vi "RemoteVI Send Tips.vi"(0 "clients":T1(array[cluster]), 5 "message":string, 7 "message sent":string) -> (4 "clients out":T1(array[cluster]), 6 "message sent out":string)   [LabVIEW 2020, in "RemoteVI.lvlib"]
doc: "Tells every client the tip strips of the panel when they changed (docs\\protocol.md 3.3): if message (RemoteVI Read Tips.vi) differs from message sent (what the clients were last told - a new client gets the current message with its greeting), it is written as a WebSocket text frame (RemoteVI WS Encode Server Frame.vi) to every client that is not closed (RemoteVI Write To Clients.vi, 500 ms per client). No VI Server call."
uses:
  RemoteVI.lvlib
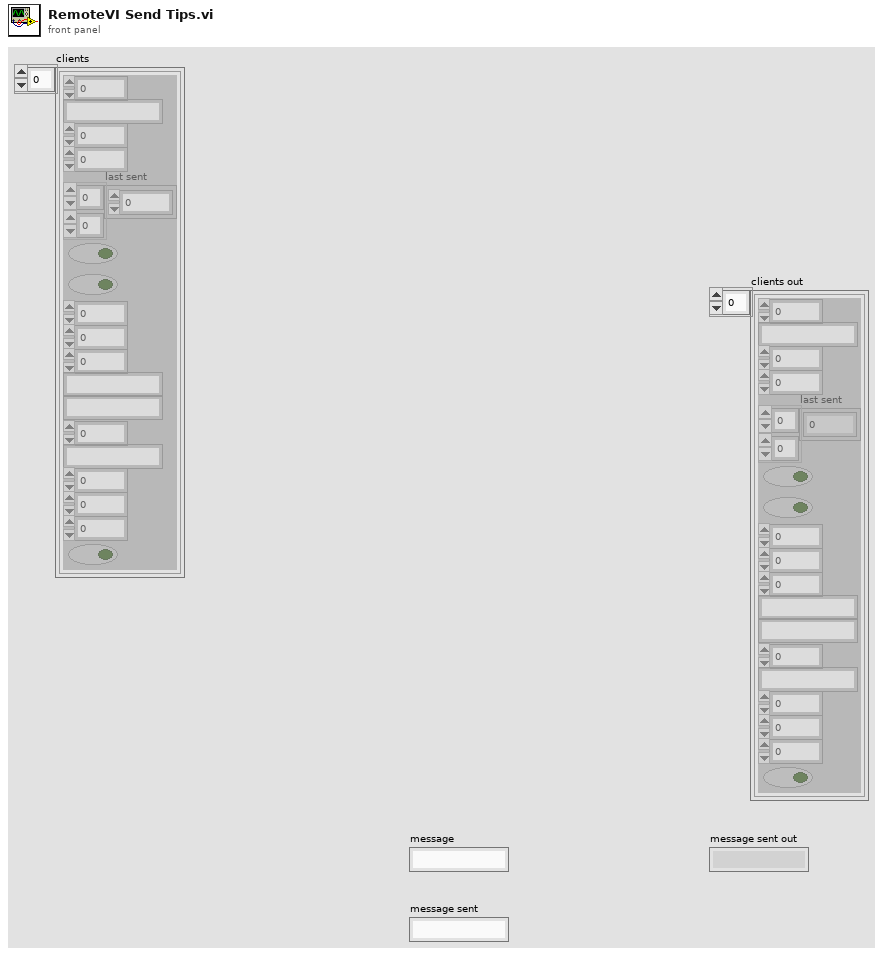
[diagram p1: front panel]
types:
  T1 = cluster{"connection":u32, "rx buffer":string, "seq":u32, "acked":u32, "last sent":u32[][], "tracking":bool, "closed":bool, "mods":u8, "mods set":u8, "popup since":u32, "windows sent":string, "window frames":cluster{"id":u64, "pixels":u32[][]}[], "key window":u64, "address":string, "since":dbl, "last input":dbl, "bytes":dbl, "view only":bool}[]
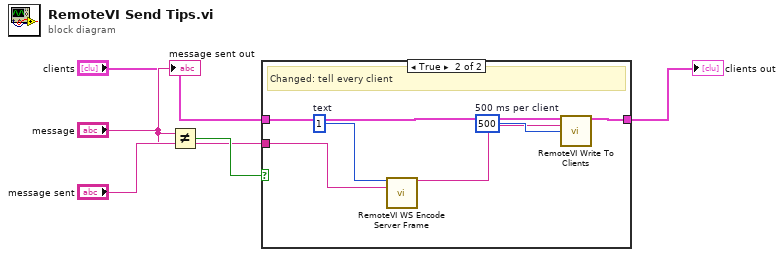
[diagram p0: block diagram]
diagram:
  n1 = Not Equal?(x="message", y="message sent") -> (x != y?=w4:bool)
  n2 = case shown="True" w4 {
    tunnel: "clients" -> [w6 w7]
    tunnel: "message" -> [_ w8]
    tunnel: [w6 w12] -> w5
    frame False {
    }
    frame True {
      w11 = 500  # 500 ms per client
      w9 = u8 1  # text
      # "Changed: tell every client"
      n3 = call "RemoteVI WS Encode Server Frame.vi"("opcode"=w9, "payload"=w8) -> ("frame"=w10:string)  [unwired: 13 in]
      n4 = call "RemoteVI Write To Clients.vi"("clients"=w7, "data"=w10, "timeout ms"=w11) -> ("clients out"=w12:T1)  [unwired: 12 in]
    }
  }
  "clients out" <- w5
  "message sent out" <- "message"
